vi "Split Log.vi"(8 "error in (no error)":errorcluster, 11 "Event Reporter Module in":refnum<class "Event Reporter Module.lvclass">) -> (0 "error out":errorcluster, 3 "Event Reporter Module out":refnum<class "Event Reporter Module.lvclass">)   [LabVIEW 2020, in "Volatus.lvlib" / "Event Reporter Module.lvclass"]
uses:
  Event Reporter Module.lvclass
  Event Reporter Module.lvclass/Event Reporter Module.ctl
  Event Level.ctl
  Volatus.lvlib
  Event.ctl
  Module/Module.lvclass
  C:/dev/lv20CE/relink/lv-volatus/Volatus/Module/Module.lvclass
  C:/dev/lv20CE/relink/lv-volatus/Volatus/Event Reporter Module/Event Reporter Module.lvclass
  VolatusAPI/VolatusAPI.lvclass
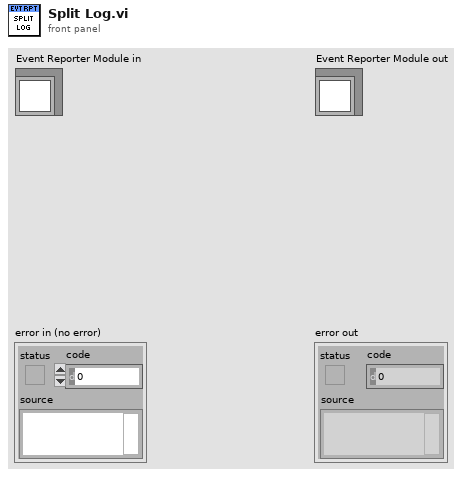
[diagram p1: front panel]
types:
  T1 = typedef "Volatus.lvlib/Event Level.ctl" = enum16{"Debug", "Info", "Warning", "Error"}
  T2 = typedef "Volatus.lvlib/Event.ctl" = cluster{"Time Stamp":timestamp, "Event Level":T1, "Context":string, "Message":string, "Error":errorcluster, "Node":string}
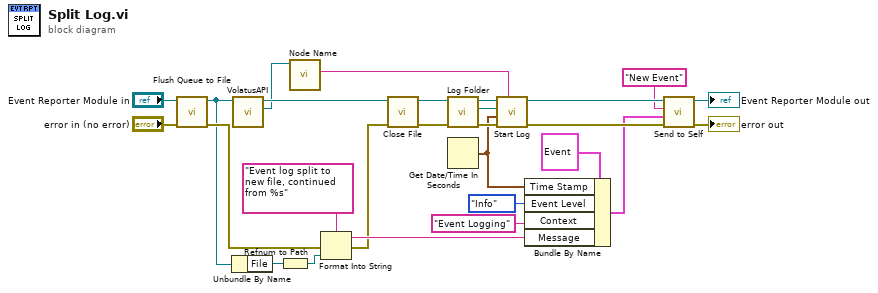
[diagram p0: block diagram]
diagram:
  n1 = call "Flush Queue to File.vi"("error in (no error)"="error in (no error)", "Event Reporter Module in"="Event Reporter Module in") -> ("error out"=w27:errorcluster, "Event Reporter Module out"=w4:refnum<class "Event Reporter Module.lvclass">)  [unwired: 8 in]
  n2 = Unbundle By Name(w4) -> ("File"=w9:refnum<file>)
  n3 = call "VolatusAPI.vi"("Module in"=w4) -> ("VolatusAPI"=w2:refnum<class "VolatusAPI.lvclass">, "Module out"=w3:refnum<class "Event Reporter Module.lvclass">)  [unwired: 9 in]
  n4 = Refnum to Path(1:w9) -> (0:w8:path)
  n5 = call "Node Name.vi"("VolatusAPI in"=w2) -> ("Node Name"=w1:string)  [unwired: 8 in, 2 out]
  n6 = Format Into String(format string="Event log split to new file, continued from %s" ("Message"), error in=w27, w8) -> (resulting string=w7:string, error out=w6:errorcluster)  [unwired: 1 in]
  n7 = call "Close File.vi"("error in (no error)"=w6, "Event Reporter Module in"=w3) -> ("error out"=w25:errorcluster, "Event Reporter Module out"=w22:refnum<class "Event Reporter Module.lvclass">)  [unwired: 8 in]
  n8 = call "Log Folder.vi"("error in (no error)"=w25, "Event Reporter Module in"=w22) -> ("error out"=w23:errorcluster, "Log Folder"=w20:path, "Event Reporter Module out"=w21:refnum<class "Event Reporter Module.lvclass">)  [unwired: 7 in]
  n9 = Get Date/Time In Seconds() -> (seconds since 1Jan1904=w12:timestamp)
  n10 = call "Start Log.vi"("Node Name"=w1, "error in (no error)"=w23, "Time Stamp"=w12, "Folder"=w20, "Event Reporter Module in"=w21) -> ("error out"=w24:errorcluster, "Event Reporter Module out"=w18:refnum<class "Event Reporter Module.lvclass">)  [unwired: 5 in]
  n11 = Bundle By Name(cluster=T2 {"Time Stamp"=timestamp(0 s since 1904-01-01), "Event Level"=enum."Info", "Context"="", "Message"="", "Error"={"status"=FALSE, "code"=0, "source"=""}, "Node"=""} ("Event"), "Time Stamp"=w12, "Event Level"=Event_Level."Info", "Context"="Event Logging", "Message"=w7) -> (w11:T2)
  n12 = call "Send to Self.vi"("error in (no error)"=w24, "Data"=w11, "Message ID"="New Event", "Module in"=w18) -> ("error out"=→"error out":errorcluster, "Module out"=→"Event Reporter Module out":refnum<class "Event Reporter Module.lvclass">)  [unwired: 6 in]
